vi "Save.vi"(8 "error in":errorcluster, 11 "Project Manager in":refnum<class "Project Manager.lvclass">) -> (0 "error out":errorcluster, 3 "Project Manager out":refnum<class "Project Manager.lvclass">)   [LabVIEW 2026, in "Project Manager.lvclass"]
doc: "Save changes to project."
uses:
  Project Manager.lvclass
  Project Manager.lvclass/Project Manager.ctl
  <vilib>/Utility/EditLVProj/Edit LVProj.lvlib
  Interfaces/ILogger/ILogger Messages/Log Msg/Log Msg.lvclass
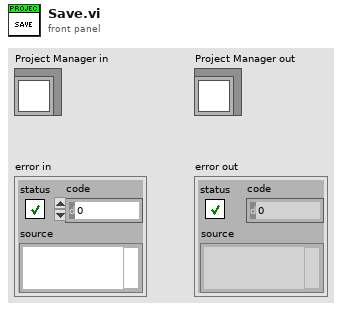
[diagram p1: front panel]
types:
  T1 = typedef "Log Entry--cluster.ctl" = cluster{"Time":timestamp, "Message":string}
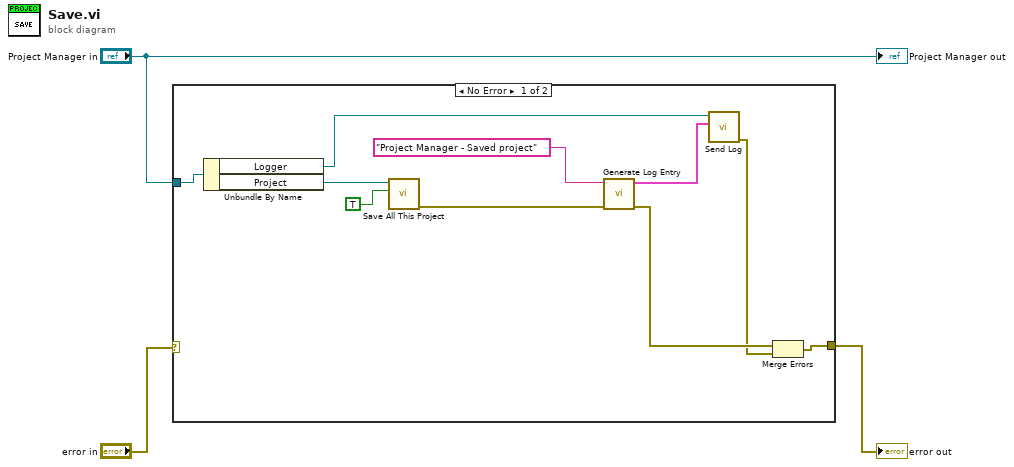
[diagram p0: block diagram]
diagram:
  n1 = case shown="No Error" "error in" {
    selector: "error in" -> [_ w14]
    tunnel: "Project Manager in" -> [w9 _]
    tunnel: [w11 w14] -> w2
    frame No Error {
      n2 = Unbundle By Name(w9) -> ("Logger"=w6:refnum<class "Message Enqueuer.lvclass">, "Project"=w8:refnum<vi>)
      n3 = call <vilib>:"Save All This Project.vi"("Exclude Dependencies? (F)"=TRUE, "Project in"=w8) -> ("error out"=w13:errorcluster)  [unwired: 8 in, 1 out]
      n4 = call "Generate Log Entry.vi"("error in"=w13, "Message"="Project Manager - Saved project") -> ("error out"=w12:errorcluster, "Log Entry"=w4:T1)  [unwired: 8 in]
      n5 = call "Send Log.vi"("Log Entry"=w4, "Message Enqueuer"=w6) -> ("error out"=w10:errorcluster)  [unwired: 8 in, 1 out]
      n6 = Merge Errors(w12, w10) -> (w11:errorcluster)
    }
    frame Error {
      # "Pass error without further action."
    }
  }
  "error out" <- w2
  "Project Manager out" <- "Project Manager in"
